vi "Data_Check.vi"(8 "error in":errorcluster, 11 "writer ref in":refnum<k21>) -> (0 "error out":errorcluster, 3 "disconnected?":bool)   [LabVIEW 2025]
uses:
  <resource>/objmgr/ni.dex.rc
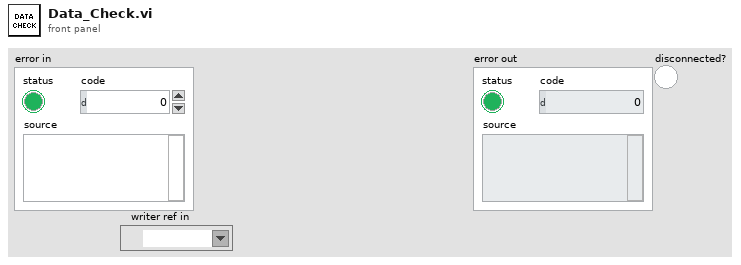
[diagram p1: front panel]
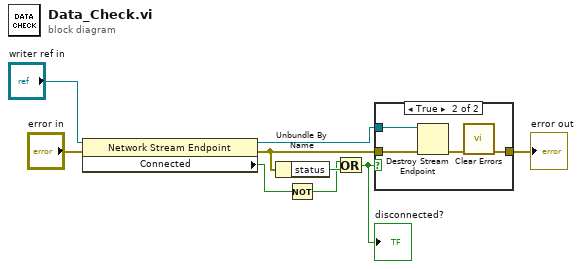
[diagram p0: block diagram]
diagram:
  n1 = property class="Network Stream Endpoint"(reference="writer ref in", error in="error in") -> (reference out=w7:refnum<k21>, error out=w6:errorcluster, "Connected"=w8:bool)
  n2 = Unbundle By Name(w6) -> ("status"=w5:bool)
  n3 = Not(x=w8) -> (.not. x?=w4:bool)
  n4 = Or(x=w4, y=w5) -> (x .or. y?=w2:bool)
  "disconnected?" <- w2
  n5 = case shown="True" w2 {
    tunnel: w7 -> [_ w14]
    tunnel: w6 -> [w10 w13]
    tunnel: [w10 w11] -> w3
    frame False {
    }
    frame True {
      n6 = Destroy Stream Endpoint(8:w13, 11:w14) -> (0:w12:errorcluster)
      n7 = call <vilib>:"Clear Errors.vi"("error in (no error)"=w12) -> ("error out"=w11:errorcluster)  [unwired: 5 in, 1 out]
    }
  }
  "error out" <- w3
